vi "Remap Resource Not Found.vi"(8 "error in":errorcluster, 10 "method":string, 11 "response":string) -> (0 "error out":errorcluster, 3 "response out":string)   [LabVIEW 2020, in "MCP Server.lvlib"]
doc: "MCP 2026-07-28 answers a resources/read for an unknown resource with error -32602 (invalid params) instead of -32002. When method is resources/read and response carries error.code -32002, response out is response with the code replaced; otherwise response out is response unchanged. Used by Complete Handler Result.vi.\n\nRuns regardless of error in, which is passed through unchanged; the JSONtext errors are not passed on."
uses:
  MCP Server.lvlib
  <vilib>/JDP Science/JSONtext/Next JSON Value.vi
  <vilib>/JDP Science/JSONtext/String Subset.vi
  <vilib>/JDP Science/JSONtext/Parsing/Advance past next JSON Value (inlined COPY).vi
  <vilib>/JDP Science/JSONtext/Parsing/Advance past whitespace.vi
  <vilib>/JDP Science/JSONtext/Parsing/Advance past String.vi
  <vilib>/JDP Science/JSONtext/Parsing/Advance past Number.vi
  <vilib>/JDP Science/JSONtext/Parsing/Advance past Line Ending.vi
  <vilib>/JDP Science/JSONtext/Parsing/Parse Full Path or Item Name.vi
  <vilib>/JDP Science/JSONtext/Parsing/Advance past Array.vi
  <vilib>/JDP Science/JSONtext/Parsing/Advance past Object.vi
  <vilib>/JDP Science/JSONtext/support/Error Cluster From Code.vi
  <vilib>/JDP Science/JSONtext/Offset/Find Item Locations by Path.vi
  <vilib>/JDP Science/JSONtext/JSONtext.lvlib
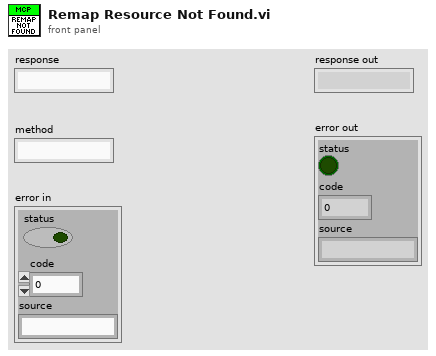
[diagram p1: front panel]
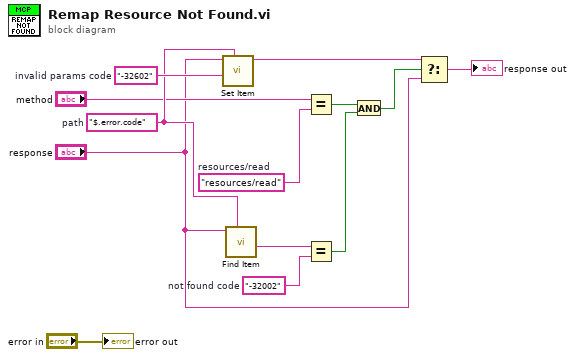
[diagram p0: block diagram]
diagram:
  w7 = "-32602"  # invalid params code
  w6 = "-32002"  # not found code
  w5 = "$.error.code"  # path
  w4 = "resources/read"  # resources/read
  n1 = call <vilib>:"Set Item.vi"("$Path or Item Name"=w5, "JSON to Insert"=w7, "JSON"="response") -> ("<JSON>"=w12:string)  [unwired: 5 in, 2 out]
  n2 = call <vilib>:"Find Item.vi"("$Path or Item Name"=w5, "JSON"="response") -> ("<JSON>"=w9:string)  [unwired: 6 in, 3 out]
  n3 = Equal?(x="method", y=w4) -> (x = y?=w8:bool)
  n4 = Equal?(x=w9, y=w6) -> (x = y?=w10:bool)
  n5 = And(x=w8, y=w10) -> (x .and. y?=w11:bool)
  n6 = Select(t=w12, s=w11, f="response") -> (s? t:f=→"response out":string)
  "error out" <- "error in"
